vi "str2str16 - MO.vi"(8 "错误输入":errorcluster, 11 "字符串":string) -> (0 "错误输出":errorcluster, 3 "string":string)   [LabVIEW 2026, in "UI-步进.lvlib"]
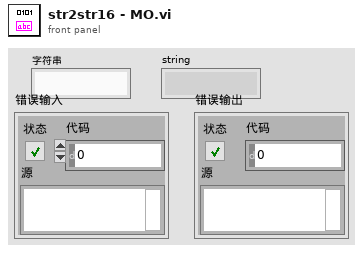
[diagram p1: front panel]
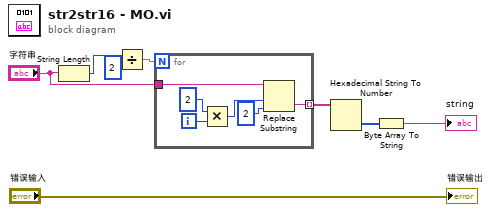
[diagram p0: block diagram]
diagram:
  n1 = String Length(string="字符串") -> (length=w2:i32)
  n2 = Divide(x=w2, y=2) -> (x/y=w4:dbl)
  n3 = for {
    N: w4 -> [_]
    tunnel: "字符串" -> [w10]
    tunnel: [w9] -> w5 mode=indexing
    i -> [w14]
    n4 = Multiply(x=2, y=w14) -> (x*y=w12:i32)
    n5 = Replace Substring(2:2 ("长度（子字符串长度）"), 3:w12, 5:w10) -> (0:w9:string)  [unwired: 1 in, 1 out]
  }
  n6 = Hexadecimal String To Number(string=w5) -> (number=w6:u32[])  [unwired: 2 in, 1 out]
  n7 = Byte Array To String(unsigned byte array=w6) -> (string=→"string":string)
  "错误输出" <- "错误输入"
